vi "Variable glob alertes Compteurs.vi"() -> ()   [LabVIEW 2022 SP3]
panel:
  out "Groupe ON":bool[](array[boolean])
  out "Liste Compteurs":string[](array[string])
  in  "groupes compteurs":T1(array[cluster]) {"valeur alerte" format="%#_6e"}
  in  "Al Compteur en cours":bool
  # "Alertes COMPTEURS"
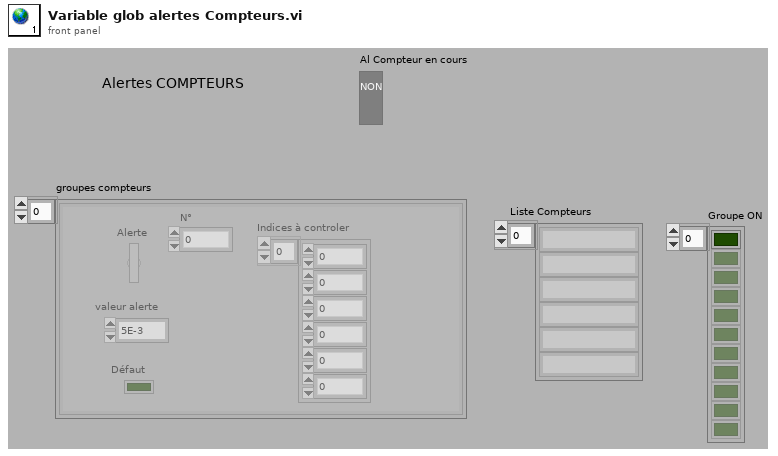
[diagram p1: front panel]
types:
  T1 = cluster{"Alerte":bool, "valeur alerte":dbl, "Défaut":bool, "Indices à controler":i16[], "N°":u16}[]
diagram:
